vi "zero position.vi"(8 "error in (no error)":errorcluster, 11 "CL57RS in":refnum<class "CL57RS.lvclass">) -> (0 "error out":errorcluster, 3 "CL57RS out":refnum<class "CL57RS.lvclass">)   [LabVIEW 2025, in "Motor.lvlib" / "CL57RS.lvclass"]
uses:
  CL57RS.lvclass
  CL57RS.lvclass/CL57RS.ctl
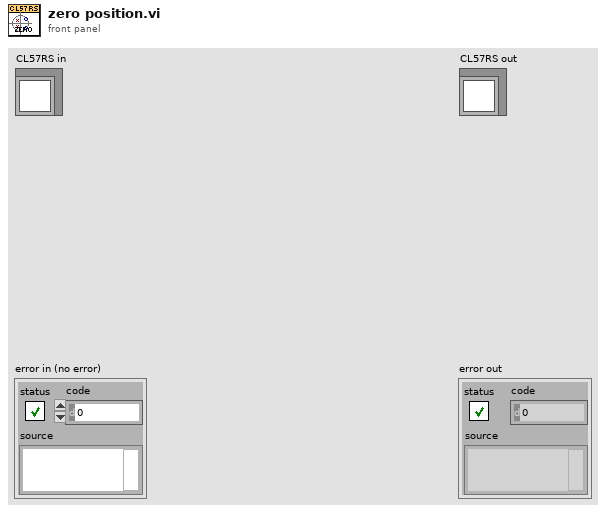
[diagram p1: front panel]
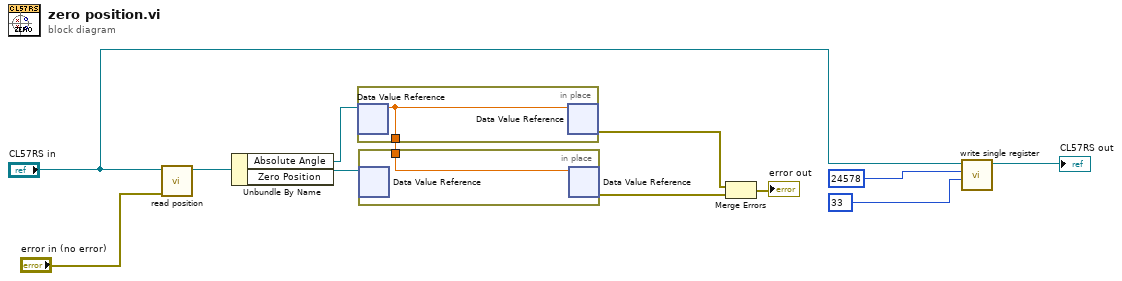
[diagram p0: block diagram]
diagram:
  n1 = call-dynamic "read position.vi"("error in (no error)"="error in (no error)", "CL57RS in"="CL57RS in") -> ("CL57RS out"=w11:refnum<class "CL57RS.lvclass">)  [unwired: 7 in, 2 out]
  n2 = Unbundle By Name(w11) -> ("Absolute Angle"=w9:refnum<data-value>, "Zero Position"=w10:refnum<data-value>)
  n3 = in-place {
    in-place-border: [w13] -> w8
    n4 = in-place-dvr #1(w9) -> (w13:dbl)  [unwired: 1 out]
    n5 = in-place-dvr #1(w13) -> (w7:errorcluster)  [unwired: 1 out]
  }
  n6 = in-place {
    in-place-border: w8 -> [w14]
    n7 = in-place-dvr #2(w10) -> ()  [unwired: 2 out]
    n8 = in-place-dvr #2(w14) -> (w6:errorcluster)  [unwired: 1 out]
  }
  n9 = Merge Errors(w7, w6) -> (→"error out":errorcluster)
  n10 = call "write single register.vi"("register to write"=u16 33 ("address"), "address"=u16 24578, "CL57RS in"="CL57RS in") -> ("CL57RS out"=→"CL57RS out":refnum<class "CL57RS.lvclass">)  [unwired: 7 in, 1 out]
